vi "PicoScope2000aSetupStreaming.vi"(0 "error in":errorcluster, 1 "Device Info":T1, 2 "handle in":i16, 3 "Acquisition Settings":T3={"Auto Stop"=FALSE, "Desired Sample Interval"=4, "Pre-trigger Samples"=0, "Post-trigger Samples"=1000, "Down-Sample Ratio"=1, "Down-Sample Mode"=0, "Time Units"=2} {"Time Units" items=["Nanoseconds (ns)"=2, "Microseconds (us)"=3, "Milliseconds (ms)"=4, "Seconds (s)"=5]; "Down-Sample Mode" items=["None"=0, "Aggregate"=1, "Decimate"=2, "Average"=4]}, 4 "Buffer and Transfer Settings":T2={"startIndex"=0, "Samples"=1000000, "Down Sample Ratio"=1, "Down-Sample Mode"=0} {"Down-Sample Mode" items=["None"=0, "Aggregate"=1, "Decimate"=2, "Average"=4]; "Down Sample Ratio" step=1; "Samples" format="%_6p"}, 5 "enabled array":i16[](array[numeric]), 10 "Pointers In":u64[][](array[numeric])) -> (11 "Pointer array":u64[][](array[numeric]), 14 "error out":errorcluster, 16 "handle out":i16, 17 "Sample Interval":u32, 19 "sampleIntervalTimeUnits":u32)   [LabVIEW 2016]
doc: "Set up the data buffers and calls RunStreaming to start the device streaming.\nData will be copied from the driver buffers into the corresponding application buffers using the wrapper dll."
uses:
  ps2000aWrap.dll
  ps2000a.dll
panel:
  # "Overview Buffer Size is the size of the temporary buffers used to\nstore data before returning it to the application."
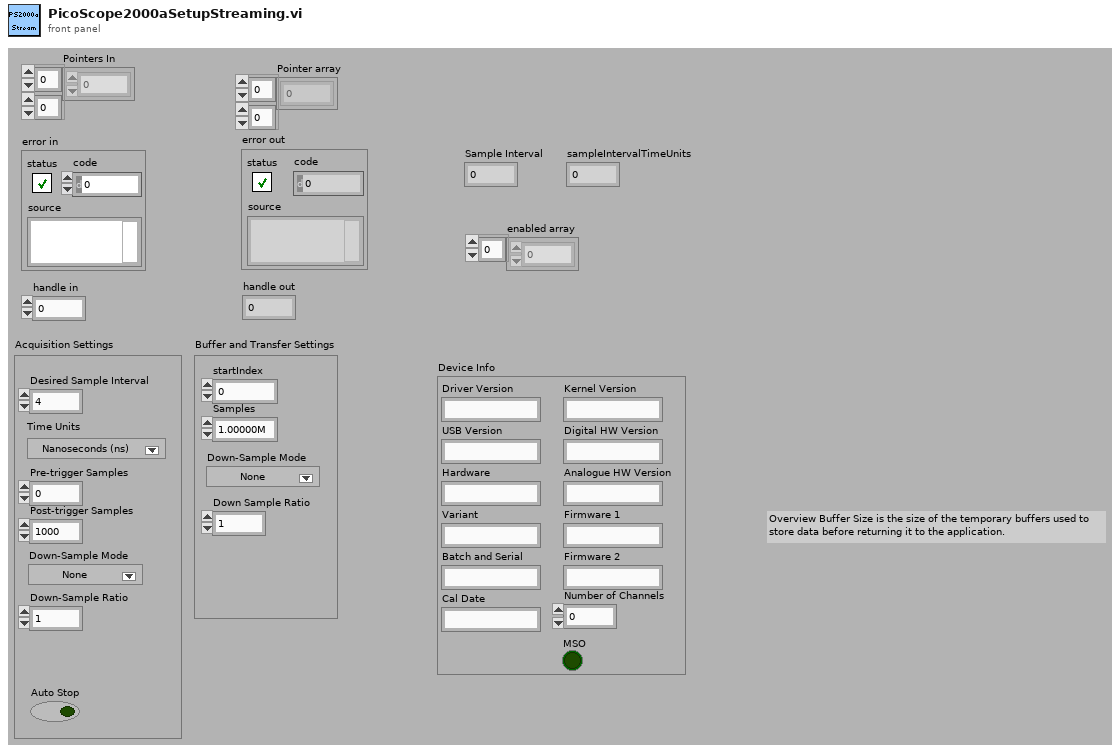
[diagram p1: front panel]
types:
  T1 = cluster{"Driver Version":string, "USB Version":string, "Hardware":string, "Variant":string, "Batch and Serial":string, "Cal Date":string, "Kernel Version":string, "Digital HW Version":string, "Analogue HW Version":string, "Firmware 1":string, "Firmware 2":string, "MSO":bool, "Number of Channels":i16}
  T2 = cluster{"startIndex":u64, "Samples":u64, "Down Sample Ratio":u64, "Down-Sample Mode":u32}
  T3 = cluster{"Auto Stop":bool, "Desired Sample Interval":u32, "Pre-trigger Samples":u32, "Post-trigger Samples":u32, "Down-Sample Ratio":u32, "Down-Sample Mode":i32, "Time Units":u32}
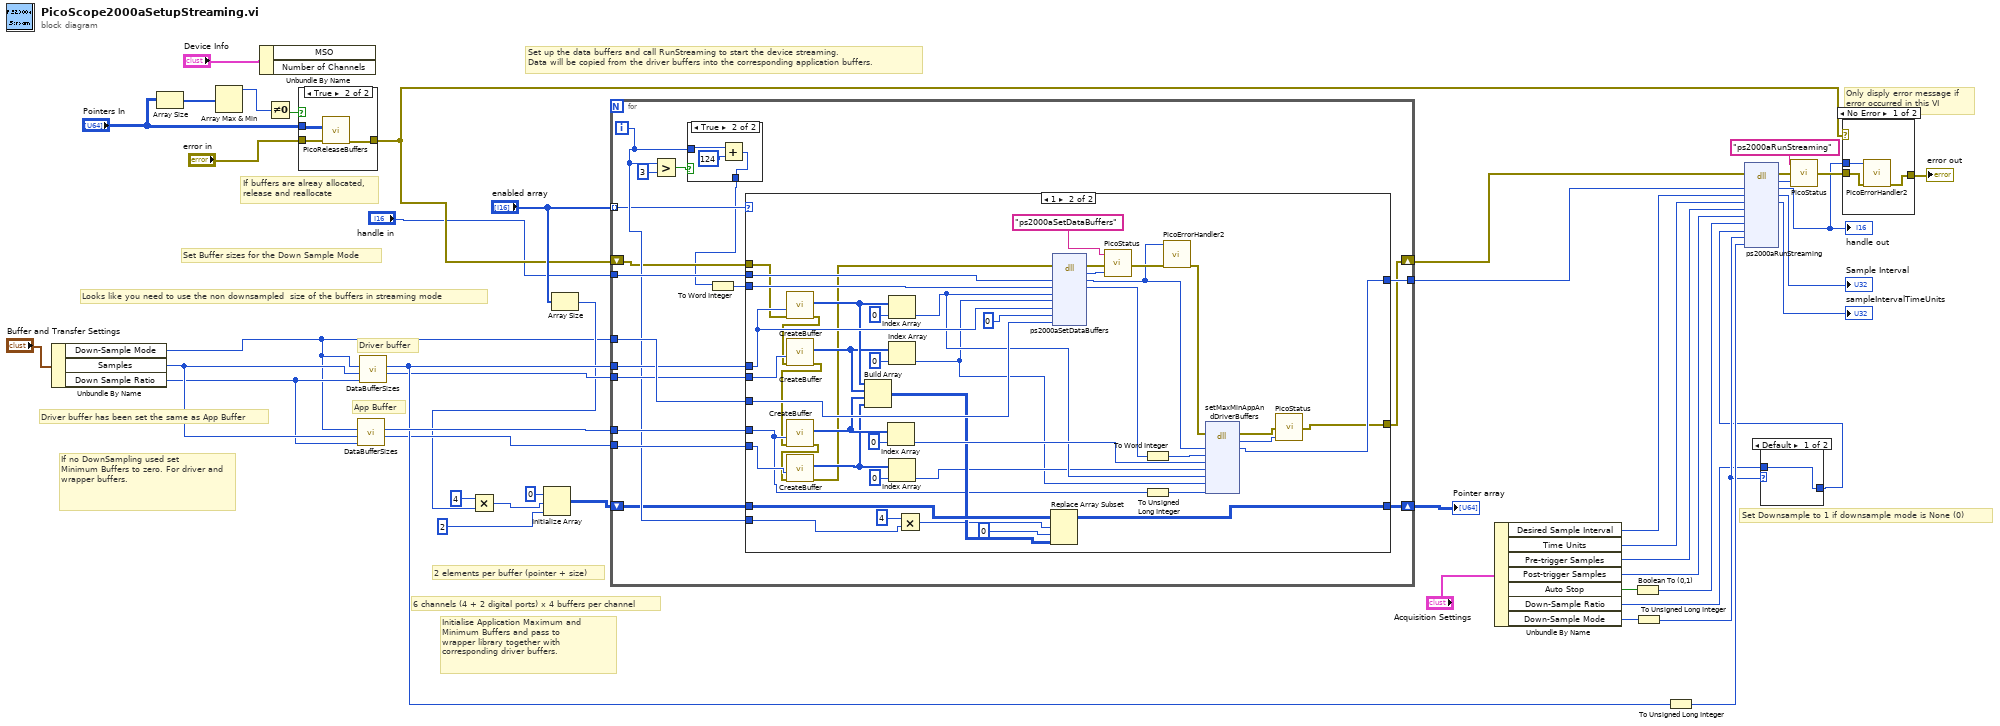
[diagram p0: block diagram]
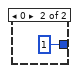
[diagram p2: hidden frame]
diagram:
  # "Set Downsample to 1 if downsample mode is None (0)"
  # "Looks like you need to use the non downsampled  size of the buffers in streaming mode"
  # "If buffers are alreay allocated,\nrelease and reallocate"
  # "2 elements per buffer (pointer + size)"
  # "6 channels (4 + 2 digital ports) x 4 buffers per channel"
  # "App Buffer"
  # "Driver buffer"
  # "Driver buffer has been set the same as App Buffer"
  # "Set Buffer sizes for the Down Sample Mode"
  # "If no DownSampling used set \nMinimum Buffers to zero. For driver and wrapper buffers."
  # "Initialise Application Maximum and\nMinimum Buffers and pass to \nwrapper library together with corresponding driver buffers."
  # "Only disply error message if\nerror occurred in this VI"
  # "Set up the data buffers and call RunStreaming to start the device streaming.\nData will be copied from the driver buffers into the corresponding application buffers."
  n1 = Unbundle By Name("Buffer and Transfer Settings") -> ("Down-Sample Mode"=w7:u32, "Samples"=w31:u64, "Down Sample Ratio"=w30:u64)
  n2 = Array Size(array="Pointers In") -> (size(s)=w10:i32[])
  n3 = Array Max & Min(array=w10) -> (max value=w9:i32)  [unwired: 3 out]
  n4 = Unbundle By Name("Device Info") -> ()  [unwired: 2 out]
  n5 = Not Equal To 0?(x=w9) -> (x != 0?=w15:bool)
  n6 = case shown="True" w15 {
    tunnel: "Pointers In" -> [_ w48]
    tunnel: "error in" -> [w47 w49]
    tunnel: [w47 w50] -> w2
    frame False {
    }
    frame True {
      n7 = call "PicoReleaseBuffers.vi"("error in (no error)"=w49, "Pointer array"=w48) -> ("error out"=w50:errorcluster)  [unwired: 9 in]
    }
  }
  n8 = call "DataBufferSizes.vi"("Down Sample Ratio"=w30, "Number of Samples"=w31, "Down-Sample Mode"=w7) -> ("min Buffer Size"=w26:i32, "Max Buffer Size"=w29:i32)  [unwired: 7 in]
  n9 = call "DataBufferSizes.vi"("Down Sample Ratio"=w30, "Number of Samples"=w31, "Down-Sample Mode"=w7) -> ("min Buffer Size"=w27:i32, "Max Buffer Size"=w28:i32)  [unwired: 7 in]
  n10 = Array Size(array="enabled array") -> (size(s)=w19:i32)
  n11 = Multiply(x=4, y=w19) -> (x*y=w20:i32)
  n12 = Initialize Array(u64 0 ("element"), w20, 2 ("dimension size")) -> (w11:u64[][])
  n13 = for {
    tunnel: "enabled array" -> [w56] mode=indexing
    tunnel: "handle in" -> [w67]
    tunnel: w7 -> [w66]
    tunnel: w29 -> [w65]
    tunnel: w28 -> [w64]
    tunnel: w27 -> [w63]
    tunnel: w26 -> [w62]
    tunnel: [w57] -> w22
    shift-right: [w55] -> w16
    shift-left: w2 -> [w54]
    shift-right: [w61] -> w25
    shift-left: w11 -> [w53]
    i -> [w58]
    n14 = Greater?(x=w58, y=3) -> (0:w59:bool)
    n15 = case shown="True" w59 {
      tunnel: [w68 w69] -> w51
      tunnel: w58 -> [w68 w71]
      frame False {
      }
      frame True {
        n16 = Add(x=w71, y=124) -> (x+y=w69:i32)
      }
    }
    n17 = To Word Integer(number=w51) -> (16bit integer=w52:i16)
    n18 = case shown="1" w56 {
      tunnel: w67 -> [w73 w119]
      tunnel: w54 -> [w72 w79]
      tunnel: w52 -> [_ w112]
      tunnel: w65 -> [_ w82]
      tunnel: w64 -> [_ w102]
      tunnel: w63 -> [_ w105]
      tunnel: w62 -> [_ w104]
      tunnel: w66 -> [_ w103]
      tunnel: w53 -> [w74 w96]
      tunnel: [w74 w95] -> w61
      tunnel: w58 -> [_ w92]
      tunnel: [w73 w88] -> w57
      tunnel: [w72 w87] -> w55
      frame 0, Default {
      }
      frame 1 {
        n19 = call "CreateBuffer.vi"("error in (no error)"=w79, "Buffer size"=w102) -> ("error out"=w78:errorcluster, "Pointer and BufferSize"=w100:u64[])  [unwired: 8 in]
        n20 = call "CreateBuffer.vi"("error in (no error)"=w78, "Buffer size"=w105) -> ("error out"=w77:errorcluster, "Pointer and BufferSize"=w99:u64[])  [unwired: 8 in]
        n21 = call "CreateBuffer.vi"("error in (no error)"=w77, "Buffer size"=w82) -> ("error out"=w76:errorcluster, "Pointer and BufferSize"=w98:u64[])  [unwired: 8 in]
        n22 = call "CreateBuffer.vi"("error in (no error)"=w76, "Buffer size"=w104) -> ("error out"=w75:errorcluster, "Pointer and BufferSize"=w97:u64[])  [unwired: 8 in]
        n23 = Build Array(w100, w99, w98, w97) -> (w91:u64[][])
        n24 = Index Array(array=w98, index=0) -> (element=w101:u64)
        n25 = Index Array(array=w100, index=0) -> (element=w94:u64)
        n26 = Index Array(array=w99, index=0) -> (element=w80:u64)
        n27 = Index Array(array=w97, index=0) -> (element=w81:u64)
        n28 = Multiply(x=4, y=w92) -> (x*y=w90:i32)
        n29 = Replace Array Subset(array=w96, new element=w91, index (row)=w90, index (col)=0 ("disabled index (row)")) -> (w95:u64[][])
        n30 = dll-call lib="ps2000a.dll" fn="ps2000aSetDataBuffers" ("ps3000.dll:_ps3000_open_unit@0")(error in=w75, "handle"=w119, "channel"=w112, "bufferMax"=w94, "bufferMin"=w80, "bufferLth"=w102, "segmentIndex"=u32 0, "downSampleRatioMode"=w103) -> (error out=w117:errorcluster, "PICO_STATUS"=w118:u32, "handle"=w84:i16, "channel"=w113:i16)  [unwired: 7 in, 1 out]
        n31 = call "PicoStatus.vi"("PICO STATUS"=w118, "error in"=w117, "source"="ps2000aSetDataBuffers") -> ("error out"=w86:errorcluster)
        n32 = To Word Integer(number=w113) -> (16bit integer=w114:i16)
        n33 = To Unsigned Long Integer(number=w82) -> (unsigned 32bit integer=w83:u32)
        n34 = call "PicoErrorHandler2.vi"("error in (no error)"=w86, "handle In"=w84) -> ("error out"=w85:errorcluster)  [unwired: 9 in]
        n35 = dll-call lib="ps2000aWrap.dll" fn="setMaxMinAppAndDriverBuffers"(error in=w85, "handle"=w84, "channel"=w114, "appMaxBuffer"=w101, "appMinBuffer"=w81, "driverMaxBuffer"=w94, "driverMinBuffer"=w80, "bufferLength"=w83) -> (error out=w111:errorcluster, "status"=w110:i16, "handle"=w88:i16)  [unwired: 8 in, 1 out]
        n36 = call "PicoStatus.vi"("PICO STATUS"=w110, "error in"=w111) -> ("error out"=w87:errorcluster)  [unwired: 1 in]
      }
    }
  }
  "Pointer array" <- w25
  n37 = Unbundle By Name("Acquisition Settings") -> ("Desired Sample Interval"=w39:u32, "Time Units"=w33:u32, "Pre-trigger Samples"=w38:u32, "Post-trigger Samples"=w37:u32, "Auto Stop"=w36:bool, "Down-Sample Ratio"=w5:u32, "Down-Sample Mode"=w34:i32)
  n38 = Boolean To (0,1)(Boolean=w36) -> (0, 1=w40:i16)
  n39 = To Unsigned Long Integer(number=w34) -> (unsigned 32bit integer=w6:u32)
  n40 = To Unsigned Long Integer(number=w28) -> (unsigned 32bit integer=w8:u32)
  n41 = case shown="Default" w6 {
    tunnel: [w120 u32 1 ("Down-Sample Ratio")] -> w4
    tunnel: w5 -> [w120 _]
    frame Default {
    }
    frame 0 {
    }
  }
  n42 = dll-call lib="ps2000a.dll" fn="ps2000aRunStreaming" ("ps5000a.dll:_ps3000_open_unit@0")(error in=w16, "handle"=w22, "sampleInterval"=w39, "sampleIntervalTimeUnits"=w33, "maxPreTriggerSamples"=w38, "maxPostTriggerSamples"=w37, "autoStop"=w40, "downSampleRatio"=w4, "downSampleRatioMode"=w6, "overviewBufferSize"=w8) -> (error out=w44:errorcluster, "PICO_STATUS"=w45:u32, "handle"=w12:i16, "sampleInterval"=→"Sample Interval":u32, "sampleIntervalTimeUnits"=→"sampleIntervalTimeUnits":u32)  [unwired: 8 in, 1 out]
  "handle out" <- w12
  n43 = call "PicoStatus.vi"("PICO STATUS"=w45, "error in"=w44, "source"="ps2000aRunStreaming") -> ("error out"=w42:errorcluster)
  n44 = case shown="No Error" w2 {
    tunnel: [w123 w125] -> w46
    tunnel: w42 -> [w124 w125]
    tunnel: w12 -> [w122 _]
    frame No Error {
      n45 = call "PicoErrorHandler2.vi"("error in (no error)"=w124, "handle In"=w122) -> ("error out"=w123:errorcluster)  [unwired: 9 in]
    }
    frame Error {
    }
  }
  "error out" <- w46
